vi "GET.vi"(6 "timeout (10000)":i32=10000, 7 "output file":path=path "", 8 "error in (no error)":errorcluster, 10 "url":string, 11 "HTTP Client reqwest in":refnum<class "HTTP Client reqwest.lvclass">) -> (0 "error out":errorcluster, 1 "body":string, 2 "headers":string, 3 "HTTP Client reqwest out":refnum<class "HTTP Client reqwest.lvclass">, 4 "status code":u32)   [LabVIEW 2020, in "HTTP Client reqwest.lvclass"]
uses:
  HTTP Client reqwest.lvclass
  HTTP Client reqwest.lvclass/HTTP Client reqwest.ctl
  RequestBuilder/RequestBuilder.lvclass
  Client/Client.lvclass
  Types/http_method_enum.ctl
  reqwest.lvlib
  Request/Request.lvclass
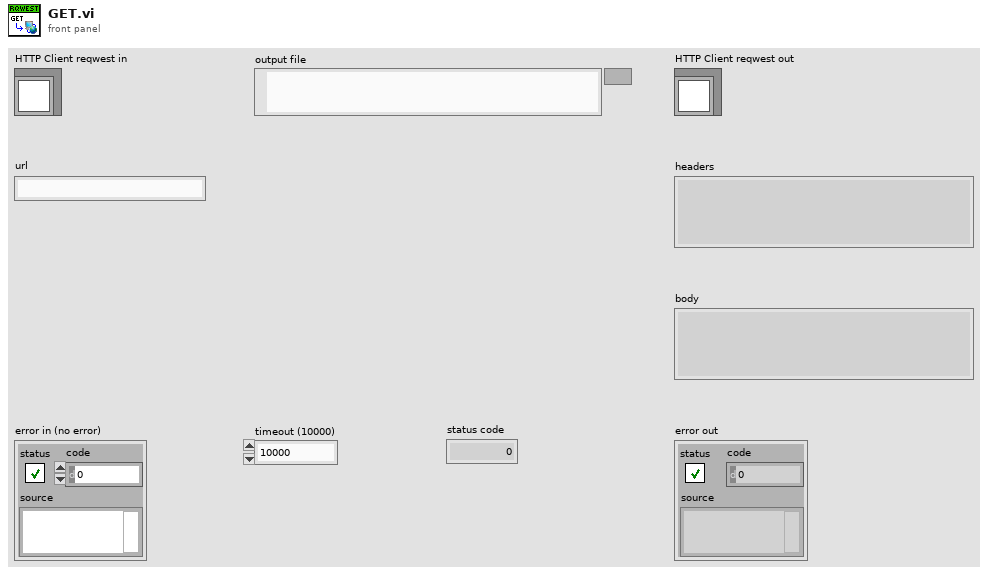
[diagram p1: front panel]
types:
  T1 = typedef "reqwest.lvlib/http_method_enum.ctl" = enum8{"<select>", "GET", "POST", "PUT", "DELETE", "HEAD", "OPTIONS", "CONNECT", "PATCH", "TRACE"}
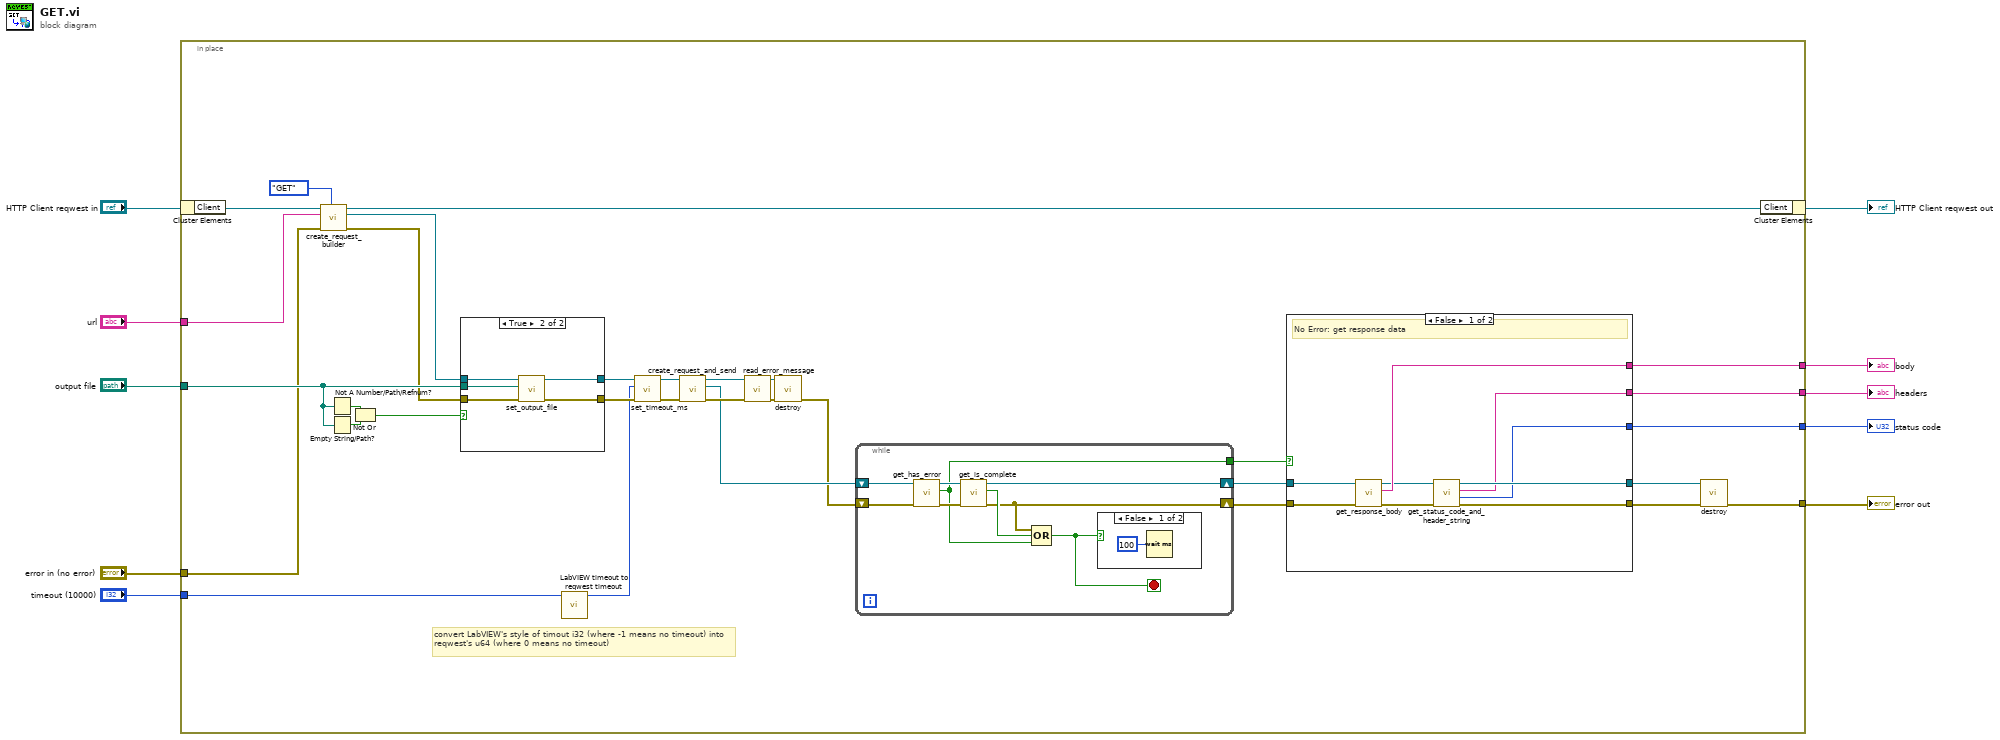
[diagram p0: block diagram]
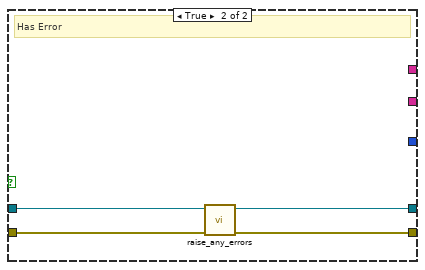
[diagram p2: hidden frame]
diagram:
  n1 = in-place {
    in-place-border: "url" -> [w40]
    in-place-border: "output file" -> [w35]
    in-place-border: "error in (no error)" -> [w34]
    in-place-border: [w22] -> w5
    in-place-border: [w20] -> w4
    in-place-border: [w19] -> w3
    in-place-border: [w12] -> w2
    in-place-border: "timeout (10000)" -> [w14]
    # "convert LabVIEW's style of timout i32 (where -1 means no timeout) into reqwest's u64 (where 0 means no timeout)"
    n2 = in-place-cluster #1("HTTP Client reqwest in") -> ("Client"=w41:refnum<class "Client.lvclass">)
    n3 = call "create_request_builder.vi"("HTTP Method"=http_method_enum."GET", "error in (no error)"=w34, "url"=w40, "Client in"=w41) -> ("error out"=w33:errorcluster, "RequestBuilder out"=w36:refnum<class "RequestBuilder.lvclass">, "Client out"=w21:refnum<class "Client.lvclass">)  [unwired: 5 in]
    n4 = Not A Number/Path/Refnum?(number/path/refnum=w35) -> (NaN/Path/Refnum?=w38:bool)
    n5 = Empty String/Path?(string/path=w35) -> (empty?=w39:bool)
    n6 = Not Or(1:w39, 2:w38) -> (0:w37:bool)
    n7 = case shown="True" w37 {
      tunnel: w36 -> [w56 w62]
      tunnel: w35 -> [_ w61]
      tunnel: [w56 w60] -> w18
      tunnel: w33 -> [w57 w59]
      tunnel: [w57 w58] -> w16
      frame False {
      }
      frame True {
        n8 = call "set_output_file.vi"("error in (no error)"=w59, "output_file"=w61, "obj in"=w62) -> ("error out"=w58:errorcluster, "obj out"=w60:refnum<class "RequestBuilder.lvclass">)  [unwired: 6 in, 1 out]
      }
    }
    n9 = call "LabVIEW timeout to reqwest timeout.vi"("-1 -> no timeout"=w14) -> ("0 -> no timeout"=w13:u64)  [unwired: 10 in]
    n10 = call "set_timeout_ms.vi"("error in (no error)"=w16, "timeout_ms"=w13, "obj in"=w18) -> ("error out"=w15:errorcluster, "obj out"=w17:refnum<class "RequestBuilder.lvclass">)  [unwired: 6 in, 1 out]
    n11 = call "create_request_and_send.vi"("error in"=w15, "obj in"=w17) -> ("error out"=w32:errorcluster, "request"=w28:refnum<class "Request.lvclass">, "obj out"=w31:refnum<class "RequestBuilder.lvclass">)  [unwired: 7 in]
    n12 = call "read_error_message.vi"("error in (no error)"=w32, "RequestBuilder in"=w31) -> ("error out"=w30:errorcluster, "RequestBuilder in"=w29:refnum<class "RequestBuilder.lvclass">)  [unwired: 7 in, 1 out]
    n13 = call "destroy.vi"("error in"=w30, "RequestBuilder in"=w29) -> ("error out"=w27:errorcluster)  [unwired: 8 in, 1 out]
    n14 = while {
      shift-right: [w66] -> w23
      shift-left: w28 -> [w70]
      shift-right: [w65] -> w24
      shift-left: w27 -> [w69]
      tunnel: [w63] -> w11
      stop <- w64 stop-if-true
      n15 = call "get_has_error.vi"("error in (no error)"=w69, "Request in"=w70) -> ("error out"=w67:errorcluster, "has_error"=w63:bool, "Request out"=w68:refnum<class "Request.lvclass">)  [unwired: 7 in]
      n16 = call "get_is_complete.vi"("error in (no error)"=w67, "Request in"=w68) -> ("error out"=w65:errorcluster, "is_complete"=w71:bool, "Request out"=w66:refnum<class "Request.lvclass">)  [unwired: 7 in]
      n17 = Compound Arithmetic op=OR(w65, w71, w63) -> (w64:bool)
      n18 = case shown="False" w64 {
        frame False {
          n19 = Wait (ms)(milliseconds to wait=u32 100) -> ()  [unwired: 1 out]
        }
        frame True {
        }
      }
    }
    n20 = case shown="False" w11 {
      tunnel: [w51 w54] -> w26
      tunnel: [w50 w55] -> w25
      tunnel: [w49 _] -> w20
      tunnel: [w48 _] -> w19
      tunnel: w23 -> [w45 w52]
      tunnel: w24 -> [w46 w53]
      tunnel: [w47 _] -> w12
      frame False {
        # "No Error: get response data"
        n21 = call "get_response_body.vi"("error in (no error)"=w46, "Request in"=w45) -> ("error out"=w43:errorcluster, "string_value"=w49:string, "Request in"=w44:refnum<class "Request.lvclass">)  [unwired: 7 in]
        n22 = call "get_status_code_and_header_string.vi"("error in (no error)"=w43, "Request in"=w44) -> ("error out"=w50:errorcluster, "status_code"=w47:u16, "headers"=w48:string, "Request out"=w51:refnum<class "Request.lvclass">)  [unwired: 6 in]
      }
      frame True {
        # "Has Error"
        n23 = call "raise_any_errors.vi"("error in (no error)"=w53, "Request in"=w52) -> ("error out"=w55:errorcluster, "Request out"=w54:refnum<class "Request.lvclass">)  [unwired: 8 in]
      }
    }
    n24 = call "destroy.vi"("error in (no error)"=w25, "Request in"=w26) -> ("error out"=w22:errorcluster)  [unwired: 8 in, 1 out]
    n25 = in-place-cluster #1("Client"=w21) -> (→"HTTP Client reqwest out":refnum<class "HTTP Client reqwest.lvclass">)
  }
  "error out" <- w5
  "headers" <- w3
  "body" <- w4
  "status code" <- w2
